vi "WriteTemplateData.vi"(8 "error in (no error)":errorcluster, 10 "Data":T1, 11 "object in":refnum<class "Template_CFG.lvclass">) -> (0 "error out":errorcluster, 3 "object out":refnum<class "Template_CFG.lvclass">)   [LabVIEW 2021, in "Template-ChannelsChild.lvlib" / "Template_CFG.lvclass"]
uses:
  Template_CFG.lvclass
  tdef/Data.ctl
  Template_CFG.lvclass/Template_CFG.ctl
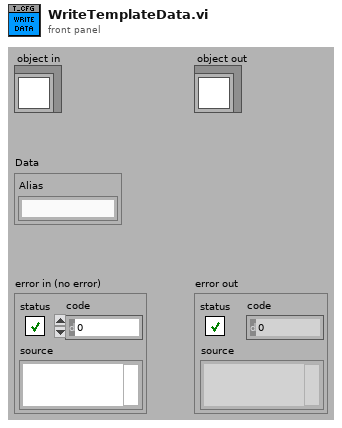
[diagram p1: front panel]
types:
  T1 = typedef "Template-ChannelsChild.lvlib/Template_CFG.lvclass/Data.ctl" = cluster{"Alias":string}
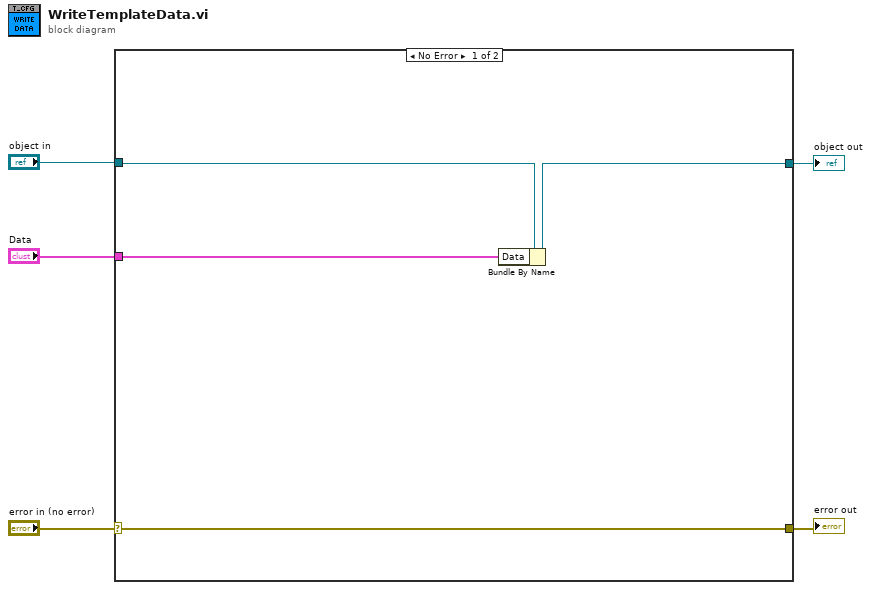
[diagram p0: block diagram]
diagram:
  n1 = case shown="No Error" "error in (no error)" {
    selector: "error in (no error)" -> [w8 w11]
    tunnel: [w8 w11] -> w4
    tunnel: [w6 w10] -> w2
    tunnel: "object in" -> [w7 w10]
    tunnel: "Data" -> [w9 _]
    frame No Error {
      n2 = Bundle By Name(cluster=w7, "Data"=w9) -> (w6:refnum<class "Template_CFG.lvclass">)
    }
    frame Error {
    }
  }
  "error out" <- w4
  "object out" <- w2
